vi "Agilent 34401 Server.vi"() -> ()   [LabVIEW 2026]
doc: "This template is for the Queued Message Handler design pattern.\n\nThe Event Handling Loop generates messages based on user interface actions.\n\nThe Message Handling Loop processes messages generated by the Event Handling Loop, or by other messages. The messages are string values, so new messages can be added easily to the Message Cases case structure in the Message Handling Loop. Each message cluster can also provide an optional value for Message Data, which is a variant that can be converted to whatever message-specific data is required."
uses:
  controls/Enums/Real or Simulation Mode.ctl
  controls/UI Data.ctl
  controls/Agilent Settings Cluster.ctl
  support/Message Queue/Enqueue Message (Single).vi
  <vilib>/Utility/error.llb/Error Cluster From Error Code.vi
  <vilib>/ErrorRing/Error Ring.xnode
  support/Message Queue/Message Queue.lvlib
  support/User Event - Stop/User Event - Stop.lvlib
  instrumentation drivers/Agilent/Agilent 34401.lvlib
panel:
  in  "Manual Range (1.00)":dbl=1.0 format="%_3f"
  in  "Enable Auto Range (F: Disable)":bool
  in  "Manual Trigger Delay (0.0 s)":dbl format="%.3f"
  in  "Enable Auto Delay (T: Enable)":bool=TRUE
  in  "Timeout (10000 ms)":u32=10000
  in  "Slope (0: Negative)":u16(ring) items=["Negative", "Positive"]
  in  "Function (0: DC Voltage)":u16(ring) items=["DC Voltage", "AC Voltage", "2 - Wire Resistance", "4 - Wire Resistance", "DC Current", "AC Current", "Frequency", "Period", "Continuity", "Diode Checking", "VDC:VDC Ratio", "Temperature", "Capacitance"]
  in  "Samples per Trigger (10)":i32=10 format="%#.6g"
  in  "Trigger Count (5)":i32=5 format="%#.6g"
  in  "Mode":T1
  in  "VISA resource name":refnum<visa-resource-name>
  out "Measurements":dbl[](graph)
  in  "Exit":bool
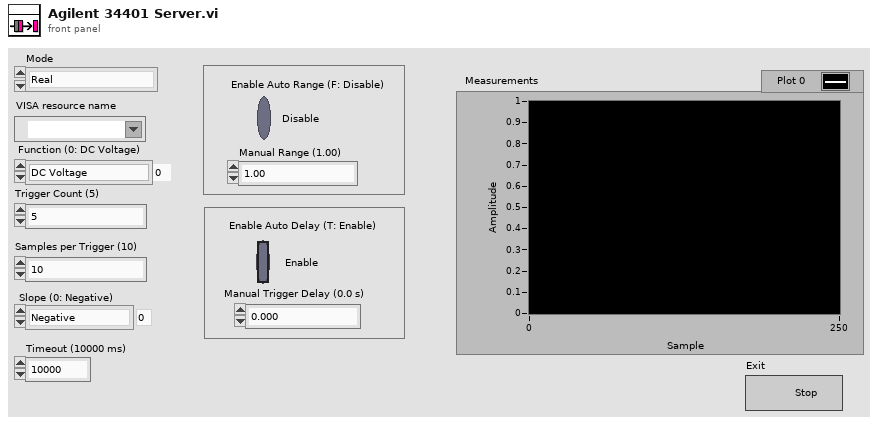
[diagram p1: front panel]
types:
  T1 = typedef "Real or Simulation Mode.ctl" = enum16{"Real", "Simulation"}
  T2 = typedef "Agilent Settings Cluster.ctl" = cluster{"Mode":T1, "VISA resource name ":refnum<visa-resource-name>, "Function (0: DC Voltage)":u16, "Trigger Count (5)":i32, "Samples per Trigger (10)":i32, "Slope (0: Negative) ":u16, "Timeout (10000 ms)":u32, "Enable Auto Range (F: Disable) ":bool, "Manual Range (1.00)":dbl, "Enable Auto Delay (T: Enable)":bool, "Manual Trigger Delay (0.0 s)":dbl}
  T3 = typedef "UI Data.ctl" = cluster{"connection ID":refnum<k5>, "Exit Button Ref":refnum<vi>}
  T4 = typedef "Message Queue.lvlib/All Message Queues.ctl" = cluster{"UI":refnum<queue>}
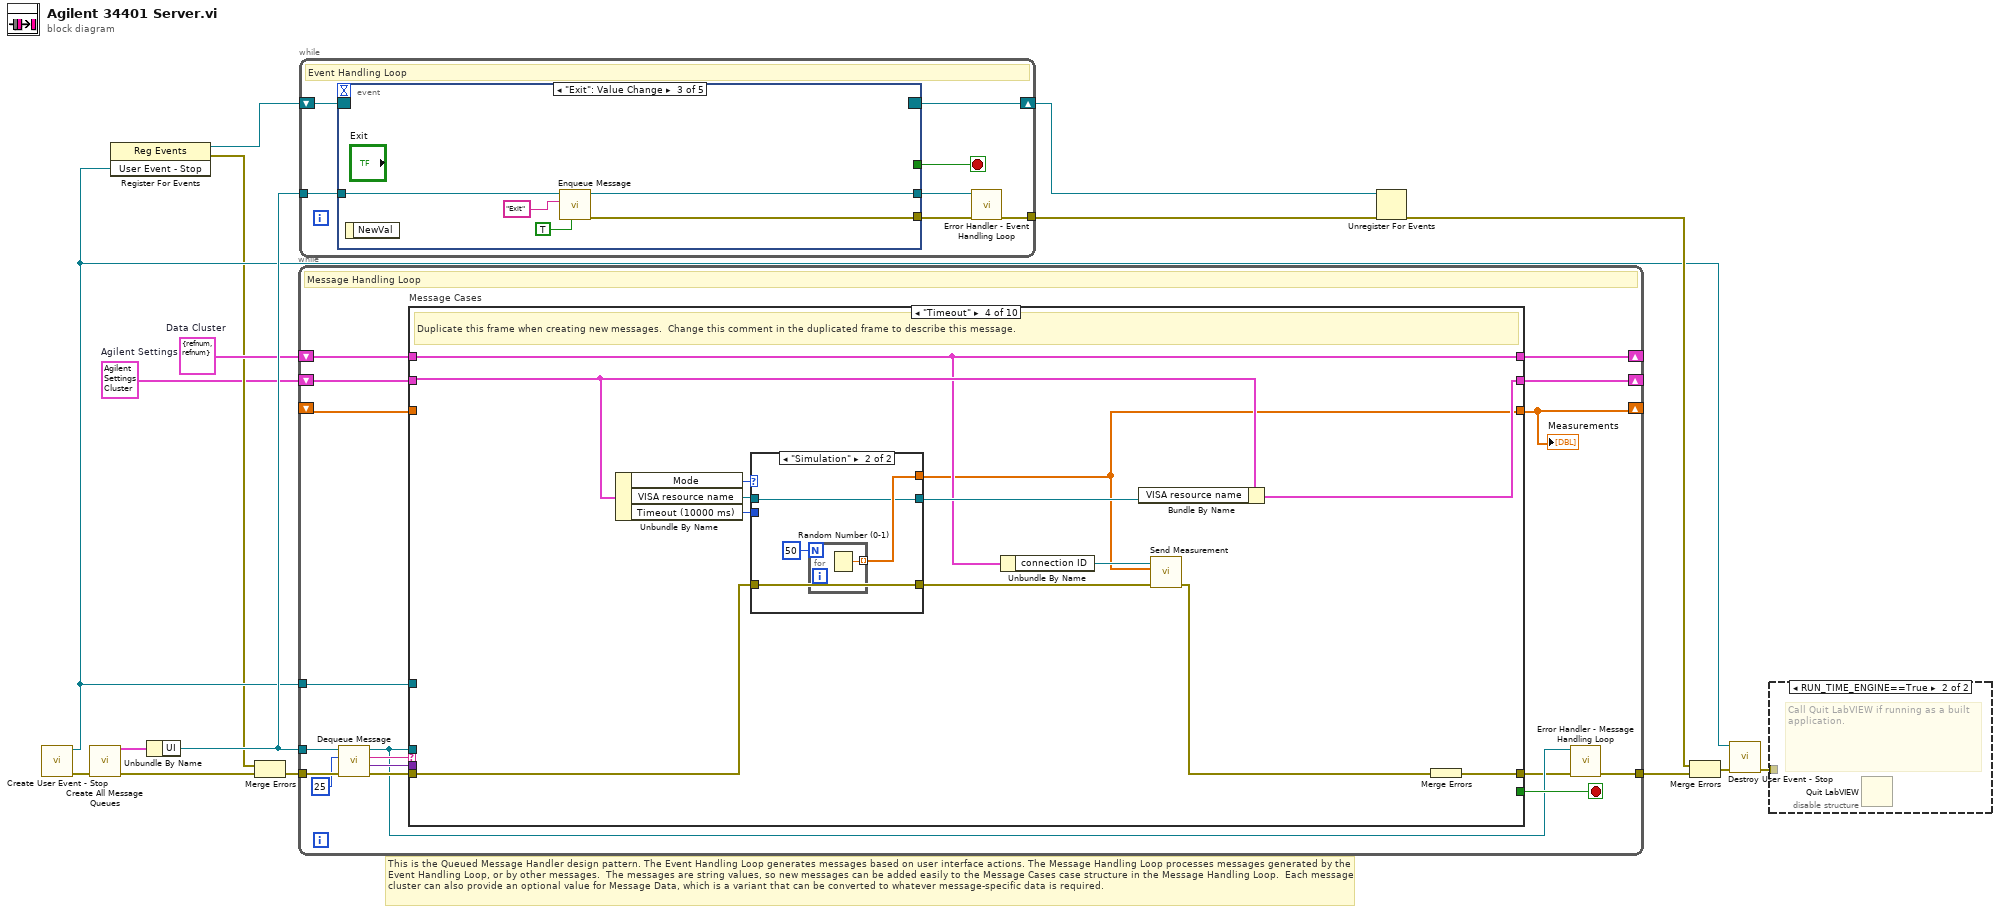
[diagram p0: block diagram]
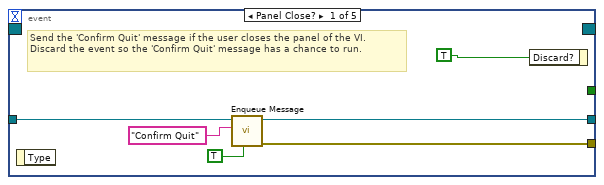
[diagram p3: hidden frame]
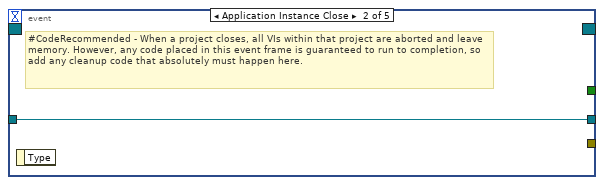
[diagram p4: hidden frame]
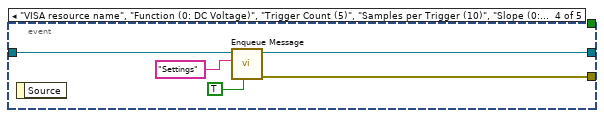
[diagram p5: hidden frame]
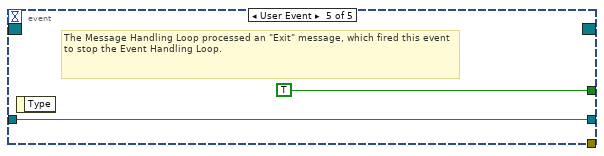
[diagram p6: hidden frame]
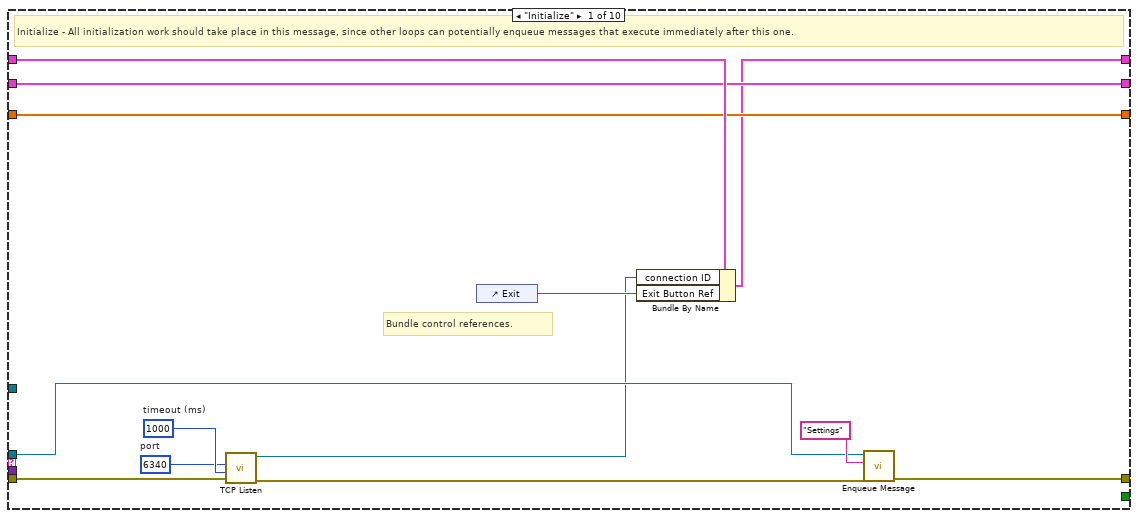
[diagram p7: hidden frame]
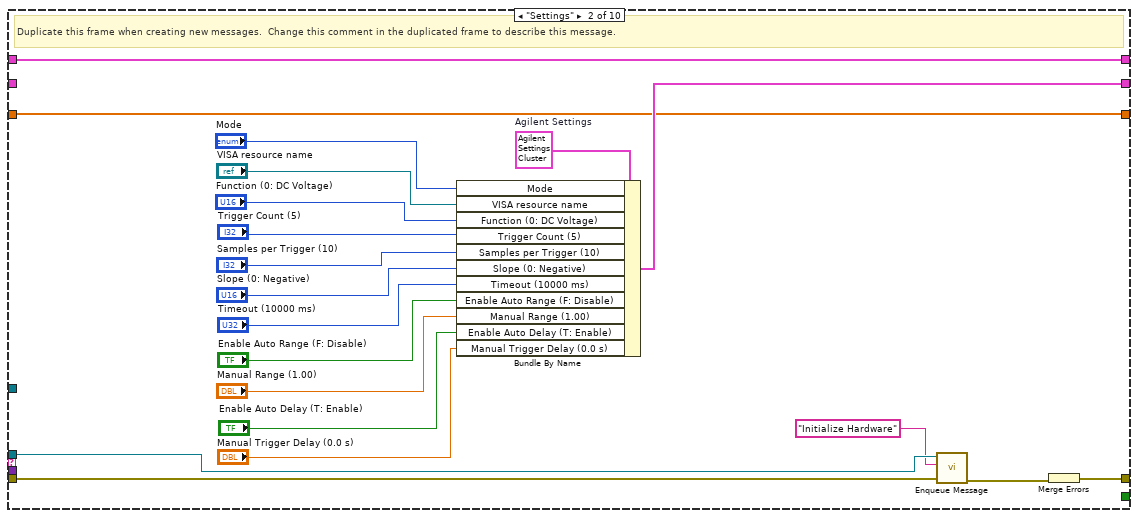
[diagram p8: hidden frame]
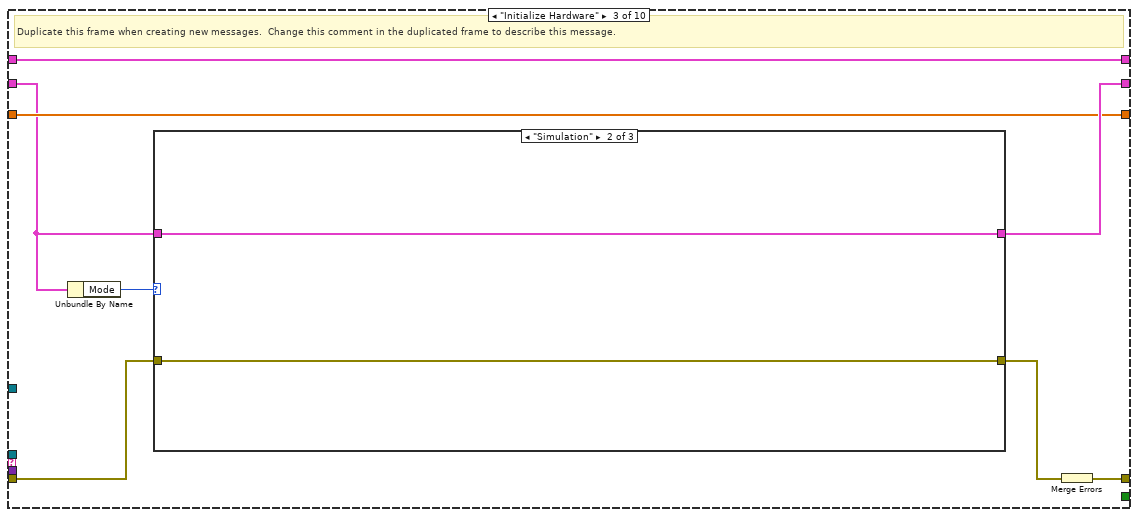
[diagram p9: hidden frame]
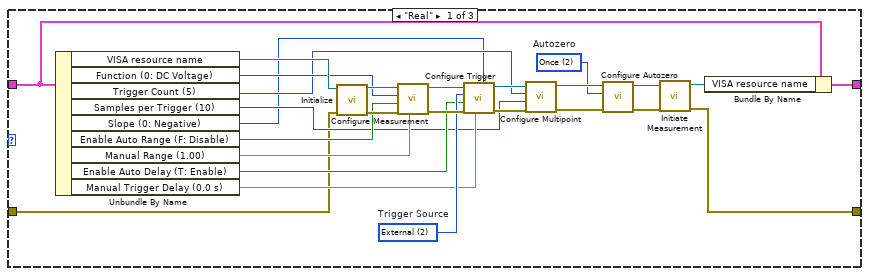
[diagram p10: hidden frame]
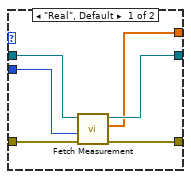
[diagram p12: hidden frame]
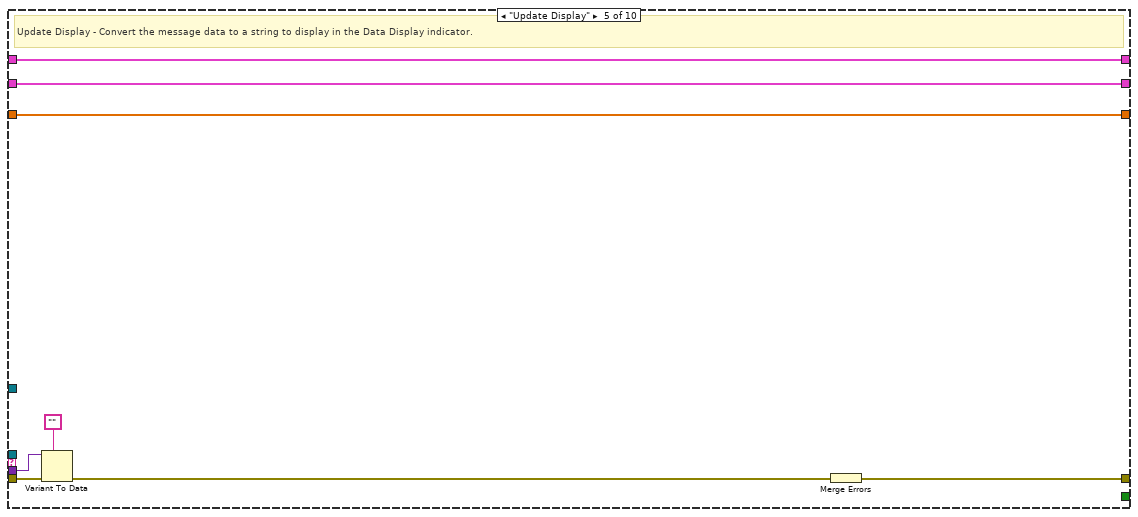
[diagram p13: hidden frame]
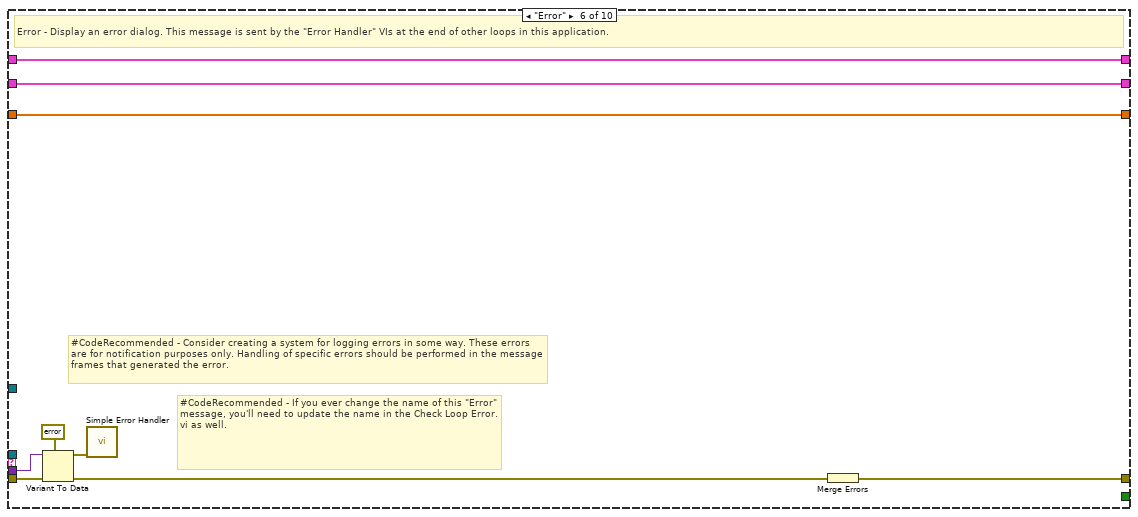
[diagram p14: hidden frame]
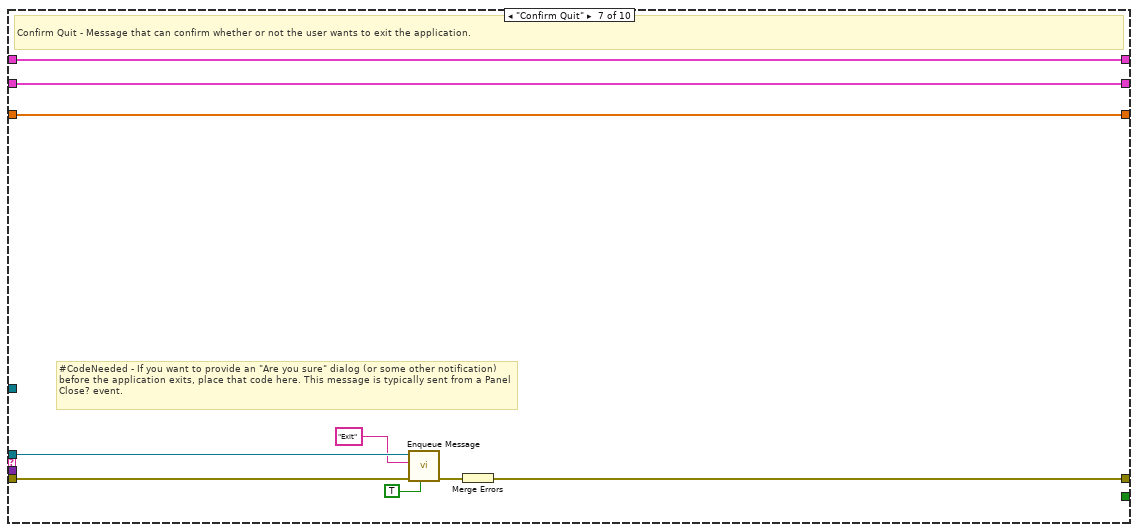
[diagram p15: hidden frame]
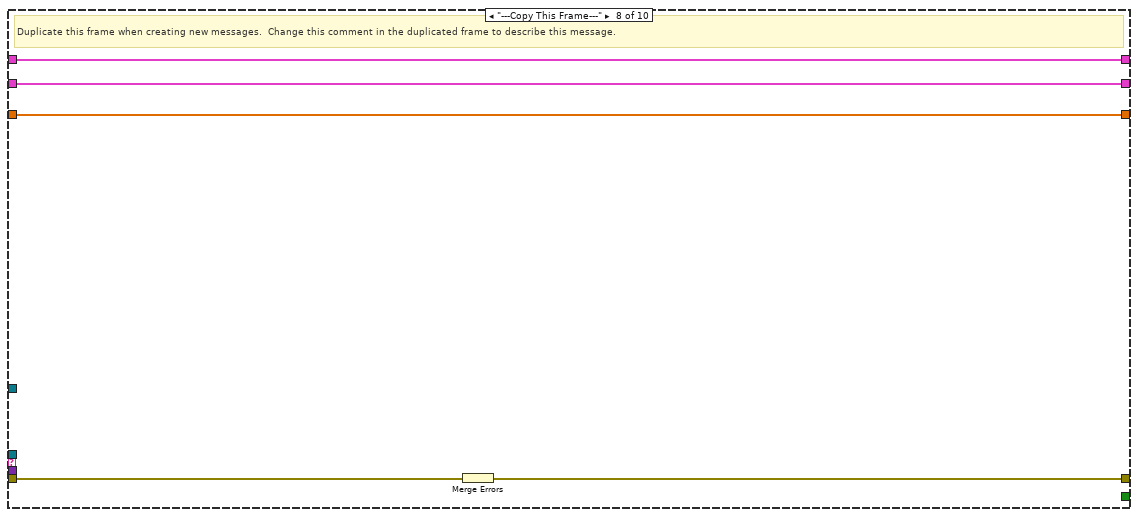
[diagram p16: hidden frame]
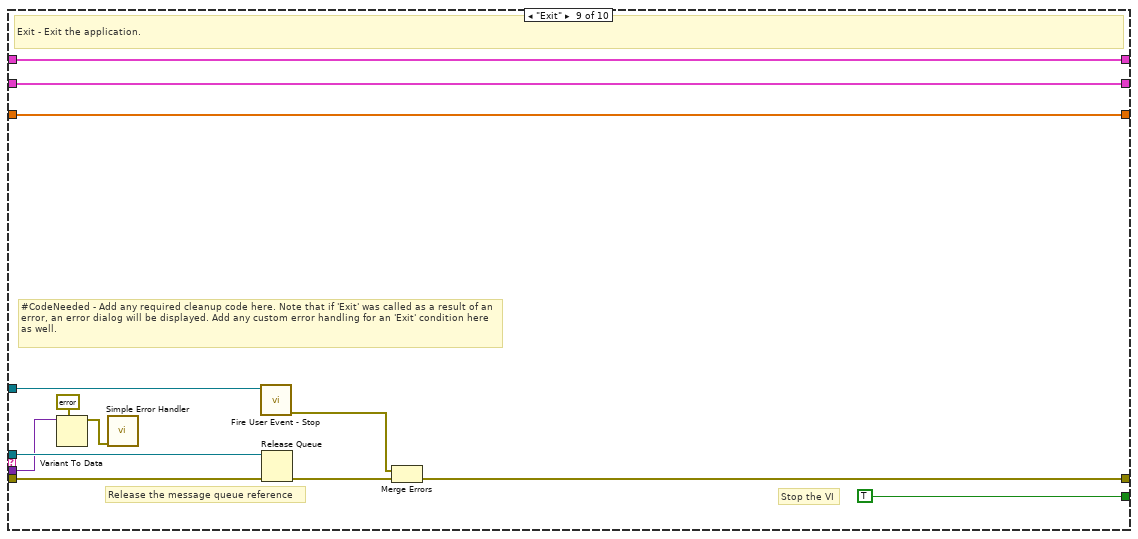
[diagram p17: hidden frame]
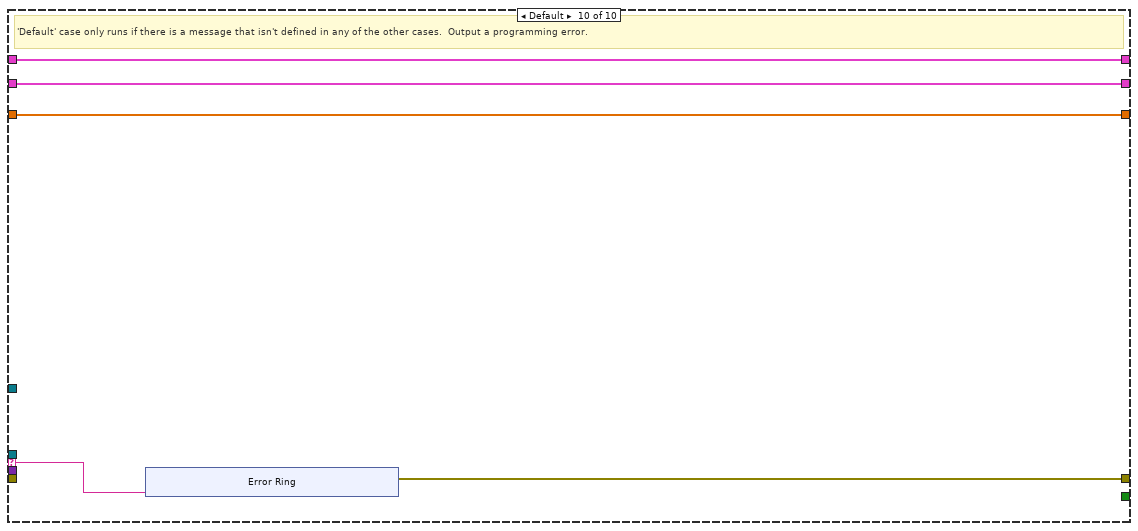
[diagram p18: hidden frame]
diagram:
  w1 = T2 {"Mode"=enum."Simulation", "VISA resource name "="", "Function (0: DC Voltage)"=0, "Trigger Count (5)"=5, "Samples per Trigger (10)"=10, "Slope (0: Negative) "=0, "Timeout (10000 ms)"=10000, "Enable Auto Range (F: Disable) "=FALSE, "Manual Range (1.00)"=1.0, "Enable Auto Delay (T: Enable)"=TRUE, "Manual Trigger Delay (0.0 s)"=0.0}  # Agilent Settings
  w8 = T3 {"connection ID"=refnum, "Exit Button Ref"=refnum}  # Data Cluster
  # "This is the Queued Message Handler design pattern. The Event Handling Loop generates messages based on user interface actions. The Message Handling Loop processes messages generated by the Event Handling Loop, or by other messages.  The messages are string values, so new messages can be added easily to the Message Cases case structure in the Message Handling Loop.  Each message cluster can also provide an optional value for Message Data, which is a variant that can be converted to whatever message-specific data is required."
  n1 = call "Create User Event - Stop.vi"() -> ("error out"=w12:errorcluster, "User Event - Stop"=w4:refnum<user-event>)  [unwired: 10 in]
  n2 = call "Create All Message Queues.vi"("error in (no error)"=w12) -> ("error out"=w16:errorcluster, "Message Queues out"=w15:T4)  [unwired: 9 in]
  n3 = register-events(w4) -> (reference out=w5:refnum<event-registration>, error out=w2:errorcluster)  [unwired: 2 in]
  n4 = Unbundle By Name(w15) -> ("UI"=w13:refnum<queue>)
  n5 = Merge Errors(w2, w16) -> (w3:errorcluster)
  n6 = while {
    tunnel: w13 -> [w25]
    shift-right: [w32] -> _
    shift-left: w8 -> [w33]
    tunnel: w4 -> [w30]
    tunnel: w3 -> [w29]
    tunnel: [w23] -> w14
    shift-right: [w21] -> _
    shift-left: w1 -> [w20]
    shift-right: [w19] -> _
    shift-left: _ -> [w18]
    stop <- w31 stop-if-true
    # "Message Handling Loop"
    n7 = call "Dequeue Message.vi"("error in (no error)"=w29, "timeout in ms (-1)"=25, "Message Queue"=w25) -> ("error out"=w28:errorcluster, "Message Data"=w26:variant, "Message"=w27:string, "dup Message Queue"=w24:refnum<queue>)  [unwired: 5 in]
    n8 = case "Message Cases" shown="\"Timeout\"" w27 {
      selector: w27 -> [_ _ _ _ _ _ _ _ _ w175]
      tunnel: w24 -> [w36 w48 _ _ _ _ w150 _ w172 _]
      tunnel: w28 -> [w38 w50 w69 w116 w134 w145 w154 w159 w165 _]
      tunnel: [w43 w53 w73 w117 w135 w139 w152 w157 w168 w176] -> w22
      tunnel: w33 -> [w46 w66 w74 w108 w136 w144 w153 w158 w171 w177]
      tunnel: [w35 w66 w74 w108 w136 w144 w153 w158 w171 w177] -> w32
      tunnel: [_ _ _ _ _ _ _ _ TRUE _] -> w31
      tunnel: w26 -> [_ _ _ _ w133 w143 _ _ w162 _]
      tunnel: w30 -> [_ _ _ _ _ _ _ _ w167 _]
      tunnel: [w44 w52 w72 w110 w130 w138 w147 w156 w161 w174] -> w21
      tunnel: w20 -> [w44 _ w68 w112 w130 w138 w147 w156 w161 w174]
      tunnel: [w41 w51 w71 w106 w129 w137 w146 w155 w160 w173] -> w19
      tunnel: w18 -> [w41 w51 w71 _ w129 w137 w146 w155 w160 w173]
      frame "Initialize" {
        w39 = u16 6340  # port
        w40 = 1000  # timeout (ms)
        # "Bundle control references."
        # "Initialize - All initialization work should take place in this message, since other loops can potentially enqueue messages that execute immediately after this one."
        n9 = call <vilib>:"TCP Listen.vi"("error in (no error)"=w38, "timeout ms (wait forever: -1)"=w40, "port"=w39) -> ("error out"=w37:errorcluster, "connection ID"=w34:refnum<k5>)  [unwired: 4 in, 3 out]
        n10 = control-ref of="Exit"() -> (w45:refnum<vi>)
        n11 = Bundle By Name(cluster=w46, "connection ID"=w34, "Exit Button Ref"=w45) -> (w35:T3)
        n12 = call-poly "Enqueue Message.vi"("error in (no error)"=w37, "Message"="Settings", "Message Queue"=w36) -> ("error out"=w43:errorcluster)  [unwired: 7 in, 1 out]
      }
      frame "Settings" {
        w65 = T2 {"Mode"=enum."Real", "VISA resource name "="", "Function (0: DC Voltage)"=0, "Trigger Count (5)"=5, "Samples per Trigger (10)"=10, "Slope (0: Negative) "=0, "Timeout (10000 ms)"=10000, "Enable Auto Range (F: Disable) "=FALSE, "Manual Range (1.00)"=1.0, "Enable Auto Delay (T: Enable)"=TRUE, "Manual Trigger Delay (0.0 s)"=0.0}  # Agilent Settings
        # "Duplicate this frame when creating new messages.  Change this comment in the duplicated frame to describe this message."
        n13 = Bundle By Name(cluster=w65, "Mode"="Mode", "VISA resource name"="VISA resource name", "Function (0: DC Voltage)"="Function (0: DC Voltage)", "Trigger Count (5)"="Trigger Count (5)", "Samples per Trigger (10)"="Samples per Trigger (10)", "Slope (0: Negative)"="Slope (0: Negative)", "Timeout (10000 ms)"="Timeout (10000 ms)", "Enable Auto Range (F: Disable)"="Enable Auto Range (F: Disable)", "Manual Range (1.00)"="Manual Range (1.00)", "Enable Auto Delay (T: Enable)"="Enable Auto Delay (T: Enable)", "Manual Trigger Delay (0.0 s)"="Manual Trigger Delay (0.0 s)") -> (w52:T2)
        n14 = call-poly "Enqueue Message.vi"("error in (no error)"=w50, "Message"="Initialize Hardware", "Message Queue"=w48) -> ("error out"=w49:errorcluster)  [unwired: 7 in, 1 out]
        n15 = Merge Errors(w49) -> (w53:errorcluster)
      }
      frame "Initialize Hardware" {
        # "Duplicate this frame when creating new messages.  Change this comment in the duplicated frame to describe this message."
        n16 = Unbundle By Name(w68) -> ("Mode"=w67:T1)
        n17 = case shown="\"Simulation\"" w67 {
          tunnel: [w78 w102 w104] -> w72
          tunnel: [w77 w101 w103] -> w70
          tunnel: w68 -> [w75 w102 w104]
          tunnel: w69 -> [w76 w101 w103]
          frame "Real" {
            w82 = u16 2 items=["On", "Off", "Once"]  # Autozero
            w92 = u16 2 items=["Immediate", "Software (Bus)", "External"]  # Trigger Source
            n18 = Unbundle By Name(w75) -> ("VISA resource name"=w99:refnum<visa-resource-name>, "Function (0: DC Voltage)"=w96:u16, "Trigger Count (5)"=w87:i32, "Samples per Trigger (10)"=w86:i32, "Slope (0: Negative)"=w85:u16, "Enable Auto Range (F: Disable)"=w97:bool, "Manual Range (1.00)"=w95:dbl, "Enable Auto Delay (T: Enable)"=w91:bool, "Manual Trigger Delay (0.0 s)"=w90:dbl)
            n19 = call "Initialize.vi"("error in (no error)"=w76, "VISA resource name"=w99) -> ("error out"=w100:errorcluster, "VISA resource name out"=w98:refnum<visa-resource-name>)  [unwired: 8 in]
            n20 = call "Configure Measurement.vi"("Manual Range (1.00)"=w95, "error in (no error)"=w100, "Enable Auto Range (T: Enable)"=w97, "Function (0: DC Voltage)"=w96, "VISA resource name"=w98) -> ("error out"=w94:errorcluster, "VISA resource name out"=w93:refnum<visa-resource-name>)  [unwired: 5 in]
            n21 = call "Configure Trigger.vi"("Slope (0: Negative)"=w85, "Manual Trigger Delay (0.0 s)"=w90, "error in (no error)"=w94, "Enable Auto Delay (T: Enable)"=w91, "Trigger Source (0: Immediate)"=w92, "VISA resource name"=w93) -> ("error out"=w89:errorcluster, "VISA resource name out"=w88:refnum<visa-resource-name>)  [unwired: 4 in]
            n22 = call "Configure Multipoint.vi"("error in (no error)"=w89, "Sample Count (1)"=w86, "Trigger Count (1)"=w87, "VISA resource name"=w88) -> ("error out"=w84:errorcluster, "VISA resource name out"=w83:refnum<visa-resource-name>)  [unwired: 6 in]
            n23 = call "Configure Autozero.vi"("error in (no error)"=w84, "Autozero  (0: On)"=w82, "VISA resource name"=w83) -> ("error out"=w81:errorcluster, "VISA resource name out"=w80:refnum<visa-resource-name>)  [unwired: 7 in]
            n24 = call "Initiate Measurement.vi"("error in (no error)"=w81, "VISA resource name"=w80) -> ("error out"=w77:errorcluster, "VISA resource name out"=w79:refnum<visa-resource-name>)  [unwired: 8 in]
            n25 = Bundle By Name(cluster=w75, "VISA resource name"=w79) -> (w78:T2)
          }
          frame "Simulation" {
          }
          frame Default {
          }
        }
        n26 = Merge Errors(w70) -> (w73:errorcluster)
      }
      frame "Timeout" {
        # "Duplicate this frame when creating new messages.  Change this comment in the duplicated frame to describe this message."
        n27 = Unbundle By Name(w112) -> ("Mode"=w115:T1, "VISA resource name"=w114:refnum<visa-resource-name>, "Timeout (10000 ms)"=w113:u32)
        n28 = case shown="\"Simulation\"" w115 {
          tunnel: [w123 w125] -> w111
          tunnel: [w122 w124] -> w109
          tunnel: w114 -> [w121 w125]
          tunnel: w116 -> [w120 w124]
          tunnel: w113 -> [w119 _]
          tunnel: [w118 w126] -> w106
          frame "Real", Default {
            n29 = call "Fetch Measurement.vi"("error in (no error)"=w120, "Timeout (10000 ms)"=w119, "VISA resource name"=w121) -> ("error out"=w122:errorcluster, "Measurements"=w118:dbl[], "VISA resource name out"=w123:refnum<visa-resource-name>)  [unwired: 5 in, 1 out]
          }
          frame "Simulation" {
            n30 = for {
              N: 50 ("# of Points") -> [_]
              tunnel: [w128] -> w126 mode=indexing
              n31 = Random Number (0-1)() -> (number: 0 to 1=w128:dbl)
            }
          }
        }
        n32 = Unbundle By Name(w108) -> ("connection ID"=w107:refnum<k5>)
        n33 = Bundle By Name(cluster=w112, "VISA resource name"=w111) -> (w110:T2)
        n34 = call "Send Measurement.vi"("error in (no error)"=w109, "Data"=w106, "TCP Network Connection in"=w107) -> ("error out"=w105:errorcluster)  [unwired: 7 in, 1 out]
        n35 = Merge Errors(w105) -> (w117:errorcluster)
      }
      frame "Update Display" {
        # "Update Display - Convert the message data to a string to display in the Data Display indicator."
        n36 = Variant To Data(error in=w134, type="", Variant=w133) -> (error out=w131:errorcluster)  [unwired: 1 out]
        n37 = Merge Errors(w131) -> (w135:errorcluster)
      }
      frame "Error" {
        # "#CodeRecommended - If you ever change the name of this \"Error\" message, you'll need to update the name in the Check Loop Error.vi as well."
        # "#CodeRecommended - Consider creating a system for logging errors in some way. These errors are for notification purposes only. Handling of specific errors should be performed in the message frames that generated the error."
        # "Error - Display an error dialog. This message is sent by the \"Error Handler\" VIs at the end of other loops in this application."
        n38 = Variant To Data(error in=w145, type=errorcluster {"status"=FALSE, "code"=0, "source"=""} ("error constant"), Variant=w143) -> (data=w141:errorcluster, error out=w140:errorcluster)
        n39 = call <vilib>:"Simple Error Handler.vi"("error in (no error)"=w141) -> ()  [unwired: 4 in, 5 out]
        n40 = Merge Errors(w140) -> (w139:errorcluster)
      }
      frame "Confirm Quit" {
        # "#CodeNeeded - If you want to provide an \"Are you sure\" dialog (or some other notification) before the application exits, place that code here. This message is typically sent from a Panel Close? event."
        # "Confirm Quit - Message that can confirm whether or not the user wants to exit the application."
        n41 = call-poly "Enqueue Message.vi"("Priority Message? (F)"=TRUE, "error in (no error)"=w154, "Message"="Exit", "Message Queue"=w150) -> ("error out"=w151:errorcluster)  [unwired: 6 in, 1 out]
        n42 = Merge Errors(w151) -> (w152:errorcluster)
      }
      frame "---Copy This Frame---" {
        # "Duplicate this frame when creating new messages.  Change this comment in the duplicated frame to describe this message."
        n43 = Merge Errors(w159) -> (w157:errorcluster)
      }
      frame "Exit" {
        # "Stop the VI"
        # "Release the message queue reference"
        # "#CodeNeeded - Add any required cleanup code here. Note that if 'Exit' was called as a result of an error, an error dialog will be displayed. Add any custom error handling for an 'Exit' condition here as well."
        # "Exit - Exit the application."
        n44 = Variant To Data(type=errorcluster {"status"=FALSE, "code"=0, "source"=""} ("error constant"), Variant=w162) -> (data=w163:errorcluster)  [unwired: 1 in, 1 out]
        n45 = call <vilib>:"Simple Error Handler.vi"("error in (no error)"=w163) -> ()  [unwired: 4 in, 5 out]
        n46 = call "Fire User Event - Stop.vi"("User Event - Stop"=w167) -> ("error out"=w166:errorcluster)  [unwired: 10 in]
        n47 = Release Queue(queue=w172, error in (no error)=w165) -> (error out=w169:errorcluster)  [unwired: 1 in, 2 out]
        n48 = Merge Errors(w166, w169) -> (w168:errorcluster)
      }
      frame Default {
        # "'Default' case only runs if there is a message that isn't defined in any of the other cases.  Output a programming error."
        n49 = xnode "Error Ring"("parameter 0"=w175) -> ("error out"=w176:errorcluster)
      }
    }
    "Measurements" <- w19
    n50 = call "Error Handler - Message Handling Loop.vi"("error in (no error)"=w22, "Message Queue"=w24) -> ("dup error in"=w23:errorcluster)  [unwired: 8 in, 1 out]
  }
  n51 = while {
    tunnel: w13 -> [w191]
    shift-right: [w189] -> w9
    shift-left: w5 -> [w190]
    tunnel: [w185] -> w6
    stop <- w187 stop-if-true
    # "Event Handling Loop"
    n52 = event shown="[2] \"Exit\": Value Change" {
      selector: w190 -> [_ _ _ _ _]
      dyn-events: [_ _ _ _ _] -> w189
      timeout: _ -> [_ _ _ _ _]
      tunnel: [_ _ _ _ TRUE ("Discard?")] -> w187
      tunnel: w191 -> [w196 w198 w203 w208 w210]
      tunnel: [w195 _ w202 w207 _] -> w188
      tunnel: [w194 w198 w201 w206 w210] -> w186
      event Panel Close? {
        # "Send the 'Confirm Quit' message if the user closes the panel of the VI. Discard the event so the 'Confirm Quit' message has a chance to run."
        n53 = event-data() -> ()  [unwired: 1 in, 1 out]
        n54 = call-poly "Enqueue Message.vi"("Priority Message? (F)"=TRUE, "Message"="Confirm Quit", "Message Queue"=w196) -> ("error out"=w195:errorcluster, "dup Message Queue"=w194:refnum<queue>)  [unwired: 7 in]
        n55 = event-data("Discard?"=TRUE) -> ()  [unwired: 1 in, 1 out]
      }
      event Application Instance Close {
        # "#CodeRecommended - When a project closes, all VIs within that project are aborted and leave memory. However, any code placed in this event frame is guaranteed to run to completion, so add any cleanup code that absolutely must happen here."
        n56 = event-data() -> ()  [unwired: 1 in, 1 out]
      }
      event "Exit": Value Change {
        n57 = event-data() -> ()  [unwired: 1 in, 1 out]
        n58 = call-poly "Enqueue Message.vi"("Priority Message? (F)"=TRUE, "Message"="Exit", "Message Queue"=w203) -> ("error out"=w202:errorcluster, "dup Message Queue"=w201:refnum<queue>)  [unwired: 7 in]
      }
      event "VISA resource name", "Function (0: DC Voltage)", "Trigger Count (5)", "Samples per Trigger (10)", "Slope (0: Negative)", "Timeout (10000 ms)", "Enable Auto Range (F: Disable)", "Manual Range (1.00)", "Enable Auto Delay (T: Enable)", "Manual Trigger Delay (0.0 s)": Value Change {
        n59 = event-data() -> ()  [unwired: 1 in, 1 out]
        n60 = call-poly "Enqueue Message.vi"("Priority Message? (F)"=TRUE, "Message"="Settings", "Message Queue"=w208) -> ("error out"=w207:errorcluster, "dup Message Queue"=w206:refnum<queue>)  [unwired: 7 in]
      }
      event User Event {
        # "The Message Handling Loop processed an \"Exit\" message, which fired this event to stop the Event Handling Loop."
        n61 = event-data() -> ()  [unwired: 1 in, 1 out]
      }
    }
    n62 = call "Error Handler - Event Handling Loop.vi"("error in (no error)"=w188, "Message Queue"=w186) -> ("dup error in"=w185:errorcluster)  [unwired: 8 in, 1 out]
  }
  n63 = Unregister For Events(event registration refnum=w9, error in=w6) -> (error out=w10:errorcluster)
  n64 = Merge Errors(w10, w14) -> (w11:errorcluster)
  n65 = call "Destroy User Event - Stop.vi"("error in (no error)"=w11, "User Event - Stop"=w4) -> ("error out"=w7:errorcluster)  [unwired: 9 in]
  n66 = disable-structure shown="RUN_TIME_ENGINE==True" {
    disable-tunnel: w7 -> [_ _]
    frame condition #0 (active) {
    }
    frame condition #1 {
      # "Call Quit LabVIEW if running as a built application."
      n67 = Quit LabVIEW() -> ()  [unwired: 1 in]
    }
  }
